vi "CIVI Query.vi"(8 "error in":errorcluster, 10 "write buffer":string, 11 "VISA Session in":refnum<visa-resource-name>) -> (0 "error out":errorcluster, 2 "read buffer":string, 3 "VISA Session out":refnum<visa-resource-name>)   [LabVIEW 2026]
doc: "Sends a SCPI query through an existing VISA session\nand reads a response of up to 4096 bytes.\nAppends LF when needed using CIVI Ensure LF.vi.\nRead termination and timeout are configured by CIVI Initialize.vi.\nDoes not open or close the session.\nReturns the response string and communication error status."
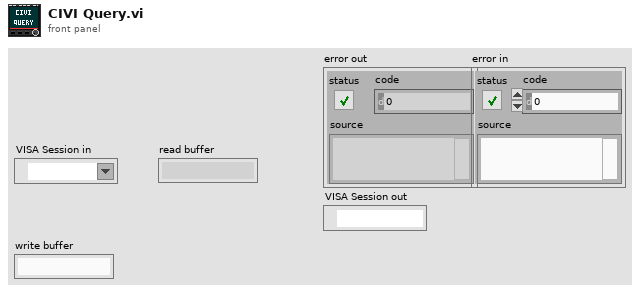
[diagram p1: front panel]
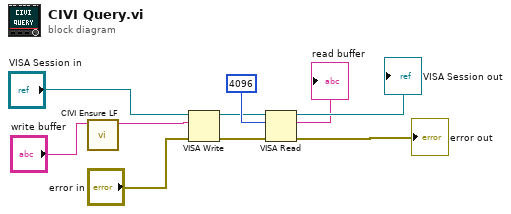
[diagram p0: block diagram]
diagram:
  n1 = call "CIVI Ensure LF.vi"("Command"="write buffer") -> ("Terminated Command"=w2:string)  [unwired: 10 in]
  n2 = VISA Write(VISA resource name="VISA Session in", write buffer=w2, error in (no error)="error in") -> (VISA resource name out=w7:refnum<visa-resource-name>, error out=w9:errorcluster)  [unwired: 1 out]
  n3 = VISA Read(VISA resource name=w7, byte count=u32 4096, error in (no error)=w9) -> (VISA resource name out=→"VISA Session out":refnum<visa-resource-name>, read buffer=→"read buffer":string, error out=→"error out":errorcluster)  [unwired: 1 out]
